vi "source.vi"() -> ()   [LabVIEW 2023]
panel:
  in  "frequency increment\n(1000Hz)":dbl=1000.0 format="%.5f"
  in  "amplitude increment\n(.1V)":dbl=0.1 format="%.5f"
  in  "source frequency\n(1000Hz)":dbl=1000.0 min=20.0 max=100000.0 format="%.5f"
  in  "output impedence\n(f:60 ohms)":bool
  in  "source amplitude\n(.6mV)":dbl=0.0006 min=0.0006 max=6.0 format="%.5f"
  out "error out":errorcluster
  in  "measurements\n(AC level)":u16(ring) items=["AC level", "DC level", "Distortion", "Distortion level", "Signal-to-Noise", "SINAD"]
  out "value read 2":dbl format="%.7f"
  in  "stop":bool
  out "Waveform Chart":dbl[](graph)
  in  "error in (no error)":errorcluster
  in  "VISA resource name":refnum<visa-resource-name>
  # "0 to 24 dB"
  # "0 to 18 dB"
  # "input range (DC only)"
  # "input range (except DC)"
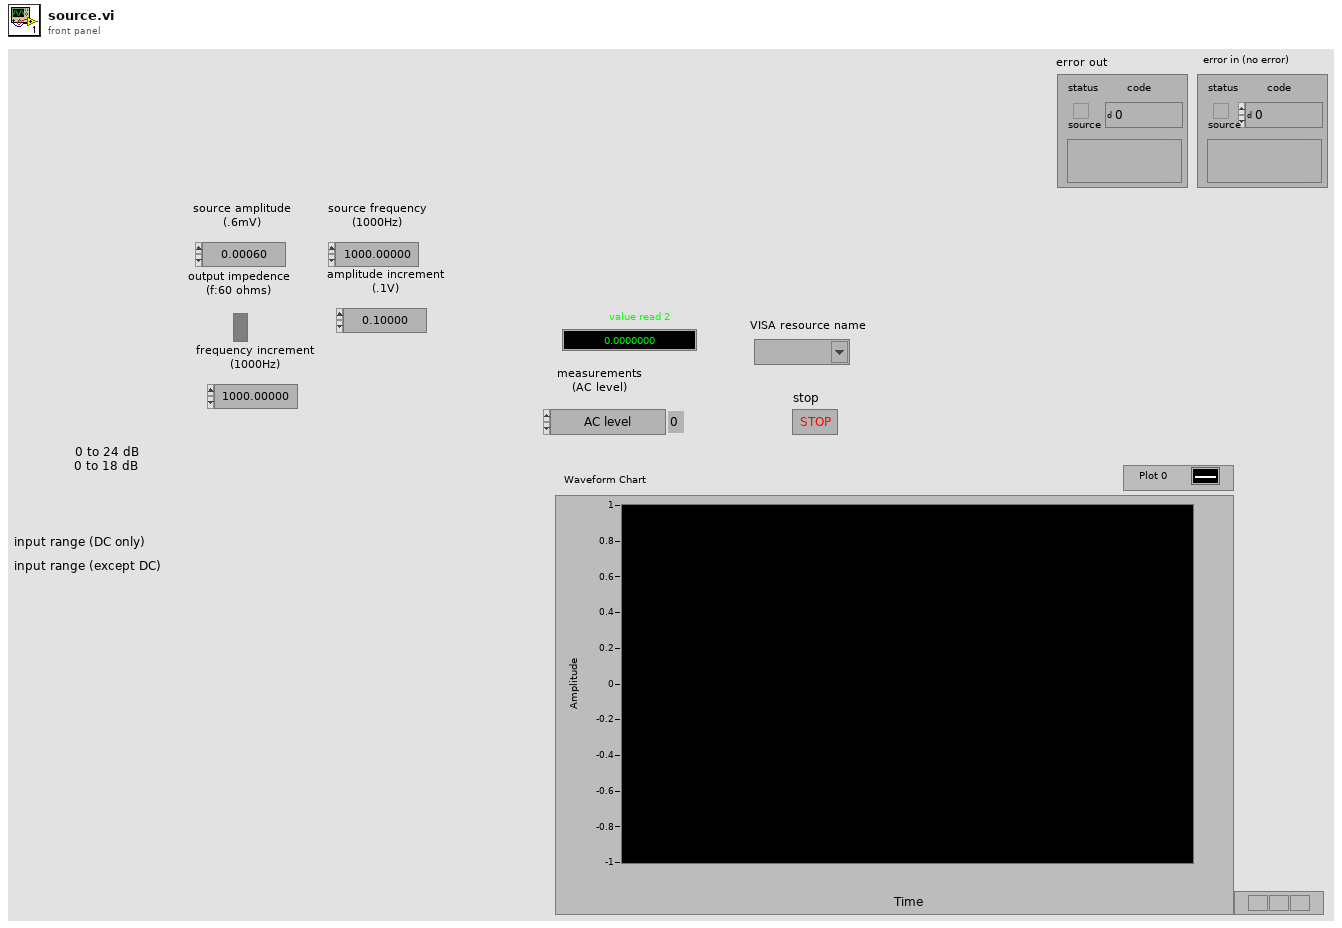
[diagram p1: front panel]
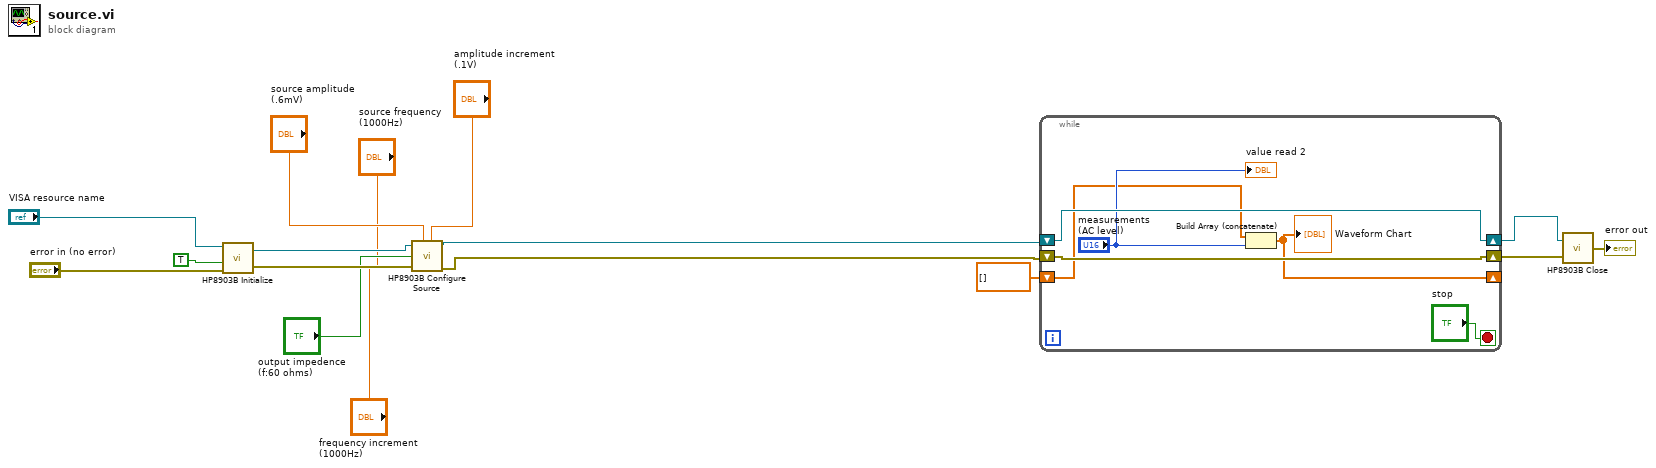
[diagram p0: block diagram]
diagram:
  n1 = call <instrlib>:"HP8903B Initialize.vi"("error in (no error)"="error in (no error)", "reset (no : F)"=TRUE, "VISA resource name"="VISA resource name") -> ("error out"=w8:errorcluster, "VISA session"=w9:refnum<visa-resource-name>)  [unwired: 1 in]
  n2 = call <instrlib>:"HP8903B Configure Source.vi"("VISA session"=w9, "source amplitude\n(.6mV)"="source amplitude\n(.6mV)", "output impedence\n(f:60 ohms)"="output impedence\n(f:60 ohms)", "error in (no error)"=w8, "source frequency\n(1000Hz)"="source frequency\n(1000Hz)", "amplitude increment\n(.1V)"="amplitude increment\n(.1V)", "frequency increment\n(1000Hz)"="frequency increment\n(1000Hz)") -> ("dup VISA session"=w7:refnum<visa-resource-name>, "error out"=w6:errorcluster)  [unwired: 2 in]
  n3 = while {
    shift-right: [w22] -> w11
    shift-left: w6 -> [w22]
    shift-right: [w21] -> w12
    shift-left: w7 -> [w21]
    shift-right: [w17] -> _
    shift-left: dbl[] [] -> [w18]
    stop <- "stop" stop-if-true
    n4 = Build Array (concatenate)(w18, "measurements\n(AC level)") -> (w17:dbl[])
    "Waveform Chart" <- w17
    "value read 2" <- "measurements\n(AC level)"
  }
  n5 = call <instrlib>:"HP8903B Close.vi"("error in (no error)"=w11, "VISA session"=w12) -> ("error out"=→"error out":errorcluster)
